vi "Write U8 FIFO.vi"(6 "FIFO Timestamps":T1, 8 "error in (no error)":errorcluster, 9 "Timeout (ms)":i32, 10 "Data in":u8[](array[numeric]), 11 "CIFFIFO in":refnum<class "CIF_Iceoryx_PCAP_Universal.lvclass">) -> (0 "error out":errorcluster, 1 "timed out?":bool, 2 "Data out":u8[](array[numeric]), 3 "CIFFIFO out":refnum<class "CIF_Iceoryx_PCAP_Universal.lvclass">)   [LabVIEW 2021, in "CIF_Iceoryx_PCAP_Universal.lvclass"]
uses:
  CIF_Iceoryx_PCAP_Universal.lvclass
  ChannelCommon/typedef/TimeStamps.ctl
  D:/dev/Packages/CIF_Channels_Core/src/CIFChannels/CIFChannels.lvclass
  CIFChannels/CIFChannels.lvclass/CIFChannels.ctl
  CIF_Iceoryx_PCAP_Universal.lvclass/CIF_Iceoryx_PCAP_Universal.ctl
  <vilib>/CIF Foundation/CIF Iceoryx/typedef/CIF Channel Header Publisher.ctl
  <vilib>/CIF Foundation/CIF Utilities/Statistics/I64/Stats_I64_CIF_U.lvclass/Stats_I64_CIF_U.ctl
  30245adb-738d-4512-91ce-9733e2d7a311.vi
  b08bf149-a330-4b4d-9064-dfddb4113935.vi
  CIFChannels/Accessors/Read FIFO Backpressure.vi
  <vilib>/CIF Foundation/CIF Utilities/Statistics/I64/X1 minus X0.vi
  <vilib>/CIF Foundation/CIF Iceoryx/SubVIs/Get Path.vi
  <vilib>/CIF Foundation/CIF Iceoryx/SubVIs/Convert Error.vi
  <vilib>/CIF Foundation/CIF Iceoryx/SubVIs/Check data length for publish.vi
  <vilib>/CIF Foundation/CIF Iceoryx/Refnum/CIF Publisher from Refnum.vi
  <vilib>/CIF Foundation/CIF Utilities/Time/System Time/LabVIEW Time to TAI Time.vi
  <vilib>/CIF Foundation/CIF Utilities/Statistics/I64/X1 minus X0.vi/dfabcf33-0dbc-4041-80a5-3dc0c86d2989.vi
  <vilib>/CIF Foundation/CIF Utilities/Statistics/I64/X1 minus X0.vi/dfabcf33-0dbc-4041-80a5-3dc0c86d2989.vi/9eb60a9a-770f-4d2d-8b3f-8465c267ecc9.vi
  <vilib>/CIF Foundation/CIF Iceoryx/PubSub/CIF pcap/Get CIF Subscriber Count.vi
  <vilib>/CIF Foundation/CIF Iceoryx/SubVIs/Convert Error Core.vi
  <vilib>/CIF Foundation/CIF Iceoryx/Iceoryx.lvlib
  CIFChannels/CIFChannels.lvclass
  <vilib>/CIF Foundation/CIF Utilities/Time/Time_CIF_U.lvlib
  D:/dev/Packages/CIF_Channels_Core/src/Iceorxy_Channels/CIF_Iceoryx_Chan/CIF_Iceoryx_Chn.lvclass
  D:/dev/Packages/CIF_Channels_Core/src/Iceorxy_Channels/PCAP_Universal/CIF_Iceoryx_PCAP_Universal.lvclass
  ChannelCommon/ChannelCommon.lvlib
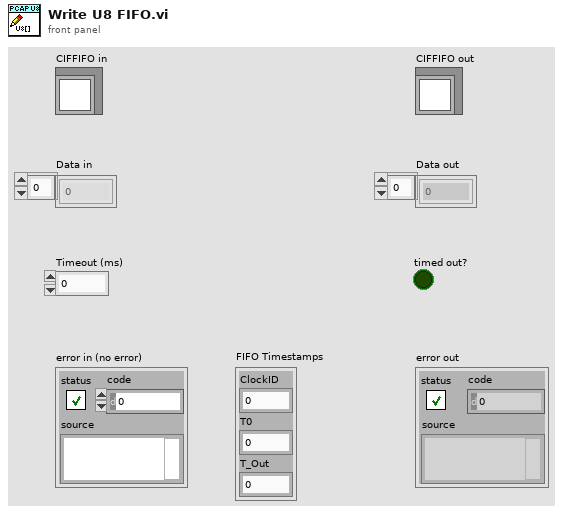
[diagram p1: front panel]
types:
  T1 = typedef "ChannelCommon.lvlib/TimeStamps.ctl" = cluster{"ClockID":u8, "T0":i64, "T_Out":i64}
  T2 = typedef "Iceoryx.lvlib/CIF Channel Header Publisher.ctl" = cluster{"T0":i64, "T_Out":i64, "T_Tx":i64, "ClockID":u8}
  T3 = typedef "Iceoryx.lvlib/CIF Publisher Refnum.ctl" = cluster{"refnum":u64, "CIF Pub":enum8{"cifpub"}}
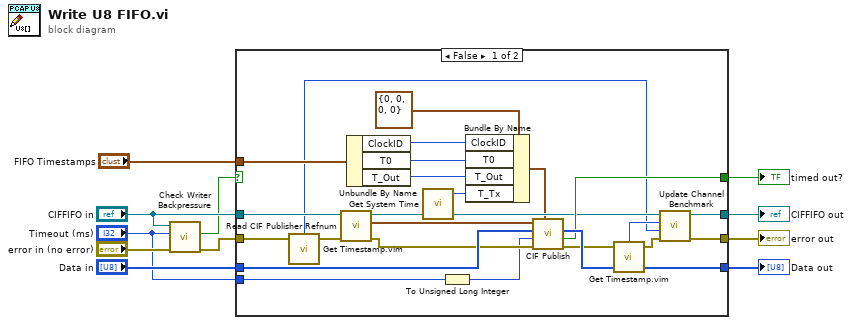
[diagram p0: block diagram]
diagram:
  n1 = call "Check Writer Backpressure.vi"("error in (no error)"="error in (no error)", "Timeout (ms)"="Timeout (ms)", "CIF_CIPC_Chn in"="CIFFIFO in") -> ("error out"=w11:errorcluster, "timed out?"=w6:bool)  [unwired: 7 in]
  n2 = case shown="False" w6 {
    selector: w6 -> [_ w37]
    tunnel: [w35 w39] -> w4
    tunnel: [w34 w36] -> w5
    tunnel: "FIFO Timestamps" -> [w27 _]
    tunnel: "Data in" -> [w33 w38]
    tunnel: "CIFFIFO in" -> [w31 w36]
    tunnel: w11 -> [w30 w39]
    tunnel: [w32 w38] -> w3
    tunnel: "Timeout (ms)" -> [w29 _]
    tunnel: [w28 w37] -> w1
    frame False {
      n3 = call "Get Timestamp.vim"("Anything in"=w30) -> ("Time (ns)"=w12:i64, "Anything out"=w19:errorcluster)  [unwired: 2 in]
      n4 = call "Read CIF Publisher Refnum.vi"("error in (no error)"=w19, "CIF_Iceoryx_PCAP_Universal in"=w31) -> ("error out"=w22:errorcluster, "CIF Publisher Refnum"=w21:T3, "CIF_Iceoryx_PCAP_Universal out"=w23:refnum<class "CIF_Iceoryx_PCAP_Universal.lvclass">)  [unwired: 7 in]
      n5 = Unbundle By Name(w27) -> ("ClockID"=w17:u8, "T0"=w15:i64, "T_Out"=w14:i64)
      n6 = call <vilib>:"Get System Time.vi"() -> ("Time (ns)"=w16:i64)  [unwired: 5 in]
      n7 = To Unsigned Long Integer(number=w29) -> (unsigned 32bit integer=w20:u32)
      n8 = Bundle By Name(cluster=T2 {"T0"=0, "T_Out"=0, "T_Tx"=0, "ClockID"=0} ("CIF Channel Header Publisher"), "ClockID"=w17, "T0"=w15, "T_Out"=w14, "T_Tx"=w16) -> (w13:T2)
      n9 = call <vilib>:"CIF Publish.vi"("CIF Channel Header Publisher"=w13, "error in (no error)"=w22, "Timeout ms"=w20, "Data In"=w33, "Publisher Reference"=w21) -> ("error out"=w24:errorcluster, "Timeout"=w28:bool, "Data Out"=w32:u8[])  [unwired: 3 in, 1 out]
      n10 = call "Get Timestamp.vim"("Anything in"=w24) -> ("Time (ns)"=w26:i64, "Anything out"=w25:errorcluster)  [unwired: 2 in]
      n11 = call "Update Channel Benchmark.vi"("error in (no error)"=w25, "X0"=w12, "X1"=w26, "CIFChannels in"=w23) -> ("error out"=w35:errorcluster, "CIFChannels out"=w34:refnum<class "CIF_Iceoryx_PCAP_Universal.lvclass">)  [unwired: 6 in]
    }
    frame True {
    }
  }
  "error out" <- w4
  "timed out?" <- w1
  "Data out" <- w3
  "CIFFIFO out" <- w5
